vi "hanwnag_OFDM_modulator 1.vi"(4 "error in (no error)":errorcluster, 5 "OFDM Parameters":T1={"FFT size (N)"=64, "Length of CP (Lc)"=8, "Null Tones"=[0, 30, 31, 32], "Training Sequence FFT size"=0, "Training Sequence Length of CP"=0, "Number of OFDM symbols (derived)"=1}, 7 "input symbols":cdb[](array[numeric])) -> (0 "error out":errorcluster, 1 "OFDM Parameters out":T1={"FFT size (N)"=64, "Length of CP (Lc)"=8, "Null Tones"=[0, 30, 31, 32], "Training Sequence FFT size"=0, "Training Sequence Length of CP"=0, "Number of OFDM symbols (derived)"=1}, 3 "output samples":cdb[](array[numeric]))   [LabVIEW 2022 SP3]
uses:
  OFDM_parameters.ctl
  <vilib>/Analysis/2dsp.llb/Inverse Complex FFT.vi
  <vilib>/Analysis/NI_AALPro.lvlib
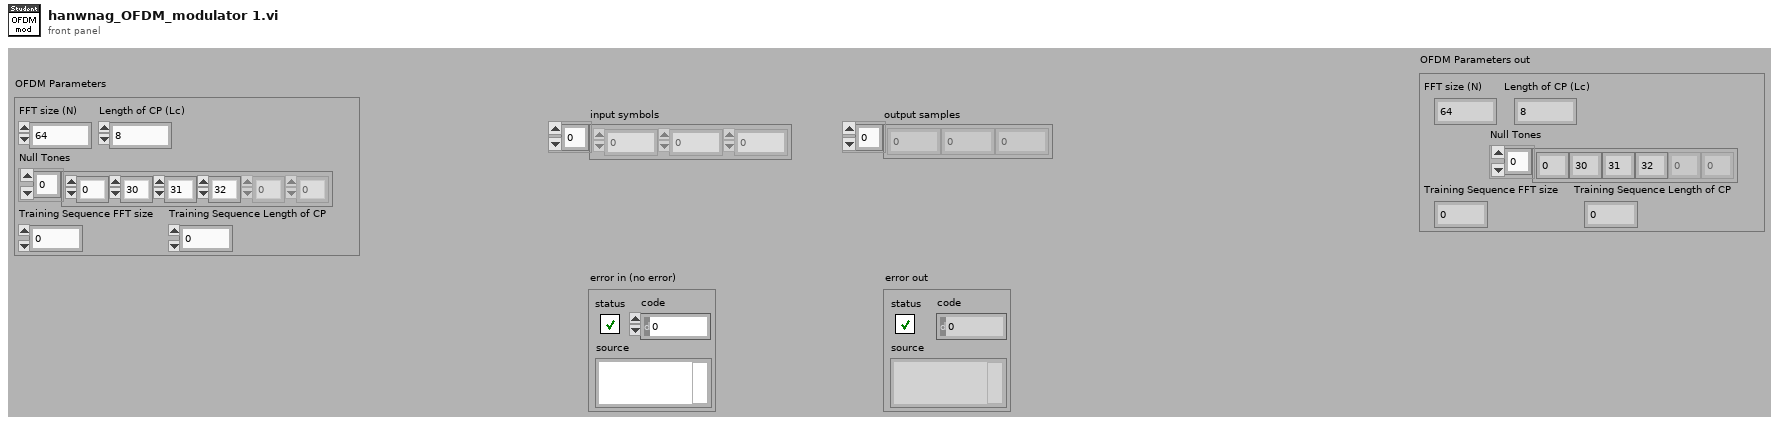
[diagram p1: front panel]
types:
  T1 = typedef "OFDM_parameters.ctl" = cluster{"FFT size (N)":i32, "Length of CP (Lc)":i32, "Null Tones":u32[], "Training Sequence FFT size":i32, "Training Sequence Length of CP":i32, "Number of OFDM symbols (derived)":i32}
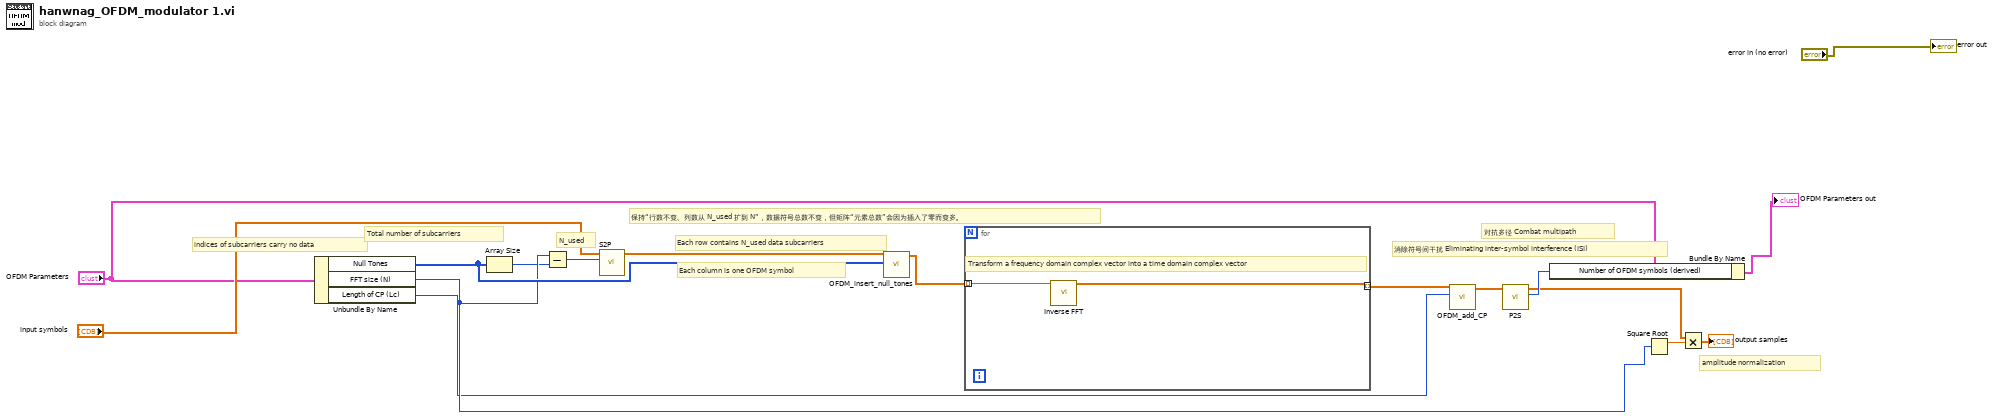
[diagram p0: block diagram]
diagram:
  # "amplitude normalization"
  # "indices of subcarriers carry no data"
  # "Each column is one OFDM symbol"
  # "消除符号间干扰 Eliminating inter-symbol interference (ISI)"
  # "对抗多径 Combat multipath"
  # "保持“行数不变、列数从 N_used 扩到 N”，数据符号总数不变，但矩阵“元素总数”会因为插入了零而变多。"
  # "Each row contains N_used data subcarriers"
  # "Total number of subcarriers"
  # "N_used"
  n1 = Unbundle By Name("OFDM Parameters") -> ("Null Tones"=w17:u32[], "FFT size (N)"=w16:i32, "Length of CP (Lc)"=w1:i32)
  n2 = Array Size(array=w17) -> (size(s)=w3:i32)
  n3 = Subtract(x=w16, y=w3) -> (x-y=w4:i32)
  n4 = call "S2P.vi"("block size"=w4, "serial input"="input symbols") -> ("parallel output"=w5:cdb[][])  [unwired: 4 in, 1 out]
  n5 = call "OFDM_insert_null_tones.vi"("null tones"=w17, "input"=w5) -> ("output"=w6:cdb[][])  [unwired: 5 in]
  n6 = for {
    tunnel: w6 -> [w19] mode=indexing
    tunnel: [w18] -> w7 mode=indexing
    # "Transform a frequency domain complex vector into a time domain complex vector"
    n7 = call-poly <vilib>:"Inverse FFT.vi"("FFT {X}"=w19) -> ("X"=w18:cdb[])  [unwired: 9 in, 1 out]
  }
  n8 = call "OFDM_add_CP.vi"("length of CP (Lc)"=w1, "input"=w7) -> ("output"=w8:cdb[][])  [unwired: 5 in]
  n9 = call "P2S.vi"("parallel input"=w8) -> ("block size"=w12:i32, "serial output"=w9:cdb[])  [unwired: 4 in, 1 out]
  n10 = Bundle By Name(cluster="OFDM Parameters", "Number of OFDM symbols (derived)"=w12) -> (→"OFDM Parameters out":T1)
  n11 = Square Root(x=w16) -> (sqrt(x)=w15:dbl)
  n12 = Multiply(x=w9, y=w15) -> (x*y=→"output samples":cdb[])
  "error out" <- "error in (no error)"
